vi "Profile_Editor.vi"(8 "error in (no error)":errorcluster={"status"=FALSE, "code"=0, "source"="\"\""}, 10 "rig envelope":string, 11 "ProfileDefinition":string) -> (0 "error out":errorcluster={"status"=FALSE, "code"=0, "source"="\"\""}, 2 "status ok":bool, 3 "Updated profile":string)   [LabVIEW 2026]
doc: "INTENT: Edit sweeps and operating points. LOGIC: Edit pressure/flow-only/combined points, ramps, controller modes, dwell and capture per point."
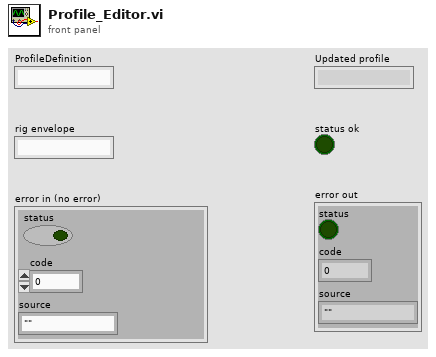
[diagram p1: front panel]
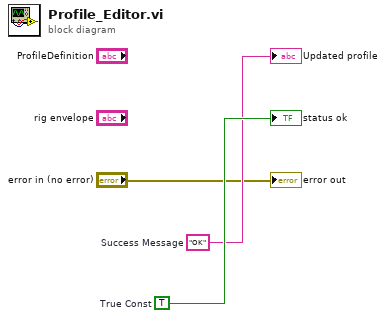
[diagram p0: block diagram]
diagram:
  w3 = TRUE  # True Const
  w2 = "OK"  # Success Message
  "Updated profile" <- w2
  "status ok" <- w3
  "error out" <- "error in (no error)"
